vi "Probe - SysAPI.vi"(8 "error in (no error)":errorcluster) -> (0 "error out":errorcluster, 1 "SysAPI Information":T2[](array[typedef]), 2 "NI Software Packages":T1[](array[typedef]))   [LabVIEW 2021, in "Acquisition.lvlib"]
doc: "Use SysAPI to detect the installed software and discovered IO devices on the running Host system. Return an array of 'Software Package's and an array of 'Host IO Resource's."
uses:
  Acquisition.lvlib
  Host IO Resource.ctl
  Host Software Package.ctl
  <vilib>/nisyscfg/Component Types.ctl
  <vilib>/nisyscfg/Get Installed Components.vi
  <vilib>/nisyscfg/Close (System).vi
  <vilib>/nisyscfg/nisyscfg.lvlib
  <resource>/objmgr/nisysapi.rc
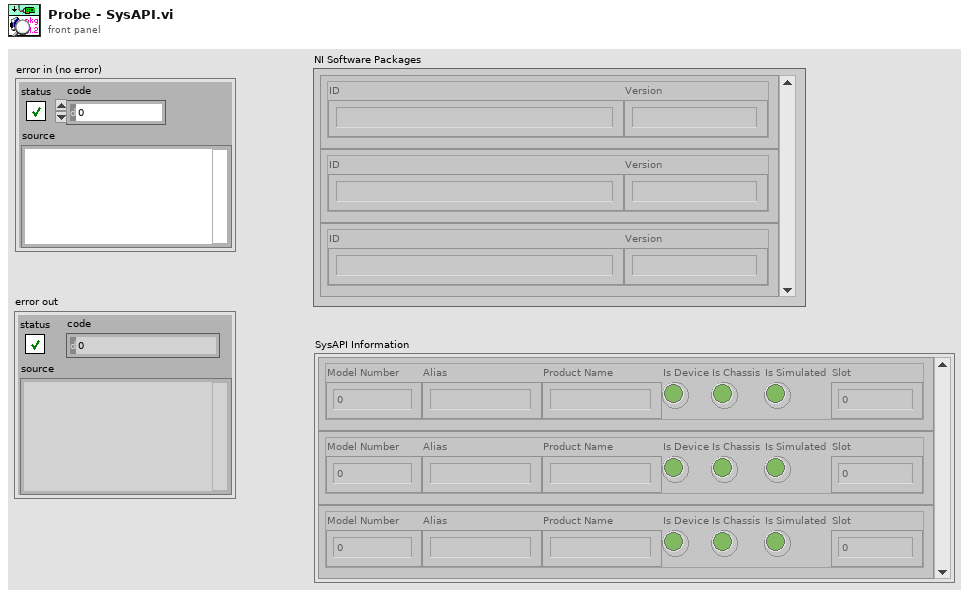
[diagram p1: front panel]
types:
  T1 = typedef "Acquisition.lvlib/Host Software Package.ctl" = cluster{"ID":string, "Version":string}
  T2 = typedef "Acquisition.lvlib/Host IO Resource.ctl" = cluster{"Model Number":u32, "Alias":string, "Product Name":string, "Is Device":bool, "Is Chassis":bool, "Is Simulated":bool, "Slot":i32}
  T3 = typedef "nisyscfg.lvlib/Component Types.ctl" = u32
  T4 = typedef "nisyscfg.lvlib/Software 1.2.ctl" = cluster{"title":string, "description":string, "ID":string, "version":string, "component type":T5}
  T5 = typedef "nisyscfg.lvlib/Component Type.ctl" = u32
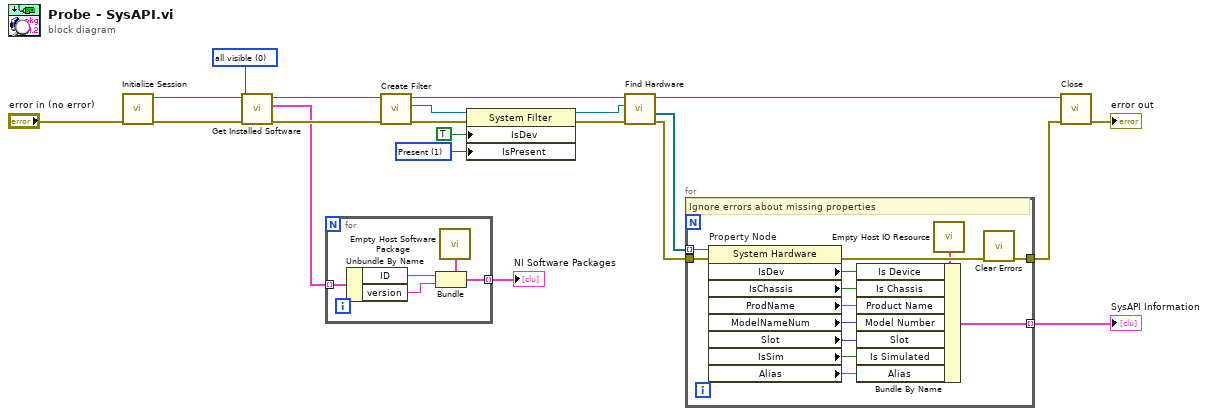
[diagram p0: block diagram]
diagram:
  w1 = 1 items=["Initializing"=-2, "Unknown"=-1, "Not Present"=0, "Present"=1] ("Devices & Chassis:Is Present")
  w17 = T3 0 items=["all visible", "all including hidden", "standard only", "startup only"] ("Item Types (all visible)")
  n1 = call <vilib>:"Initialize Session.vi"("error in (no error)"="error in (no error)") -> ("error out"=w8:errorcluster, "Session out"=w18:refnum<k21>)  [unwired: 9 in]
  n2 = call-poly <vilib>:"Get Installed Software.vi"("error in (no error)"=w8, "Item Types (all visible)"=w17, "Session in"=w18) -> ("error out"=w16:errorcluster, "Software Components"=w7:T4[], "Session out"=w15:refnum<k21>)  [unwired: 6 in]
  n3 = for {
    tunnel: w7 -> [w26] mode=indexing
    tunnel: [w24] -> w6 mode=indexing
    n4 = Unbundle By Name(w26) -> ("ID"=w23:string, "version"=w25:string)
    n5 = call "Empty Host Software Package.vi"() -> ("Software Package"=w22:T1)
    n6 = Bundle(cluster=w22, "ID"=w23, "Version"=w25) -> (w24:T1)
  }
  "NI Software Packages" <- w6
  n7 = call <vilib>:"Create Filter.vi"("error in (no error)"=w16, "Session in"=w15) -> ("error out"=w12:errorcluster, "Filter out"=w14:refnum<k20>, "Session out"=w13:refnum<k21>)  [unwired: 7 in]
  n8 = property on="Property Node" class="System Filter"(reference=w14, error in=w12, "IsDev"=TRUE ("Is Device"), "IsPresent"=w1) -> (reference out=w10:refnum<k20>, error out=w11:errorcluster)
  n9 = call <vilib>:"Find Hardware.vi"("error in (no error)"=w11, "Filter in"=w10, "Session in"=w13) -> ("error out"=w4:errorcluster, "Resources out"=w19:refnum<k20>[], "Session out"=w20:refnum<k21>)  [unwired: 5 in, 1 out]
  n10 = for {
    tunnel: w19 -> [w39] mode=indexing
    tunnel: w4 -> [w38]
    tunnel: [w36] -> w3
    tunnel: [w27] -> w2 mode=indexing
    # "Ignore errors about missing properties"
    n11 = property on="Property Node" class="System Hardware"(reference=w39, error in=w38) -> (error out=w37:errorcluster, "IsDev"=w28:bool, "IsChassis"=w29:bool, "ProdName"=w30:string, "ModelNameNum"=w31:u32, "Slot"=w32:i32, "IsSim"=w33:bool, "Alias"=w34:string)  [unwired: 1 out]
    n12 = call "Empty Host IO Resource.vi"() -> ("Host IO Resource"=w35:T2)
    n13 = Bundle By Name(cluster=w35, "Is Device"=w28, "Is Chassis"=w29, "Product Name"=w30, "Model Number"=w31, "Slot"=w32, "Is Simulated"=w33, "Alias"=w34) -> (w27:T2)
    n14 = call <vilib>:"Clear Errors.vi"("error in (no error)"=w37) -> ("error out"=w36:errorcluster)  [unwired: 5 in, 1 out]
  }
  "SysAPI Information" <- w2
  n15 = call-poly <vilib>:"Close.vi"("error in (no error)"=w3, "Session in"=w20) -> ("error out"=→"error out":errorcluster)  [unwired: 9 in]
